vi "IsUserInputInRange.vi"(11 "User Input in":T1) -> (3 "InRange?":bool)   [LabVIEW 2017]
uses:
  Ctrl/UserInput.ctl
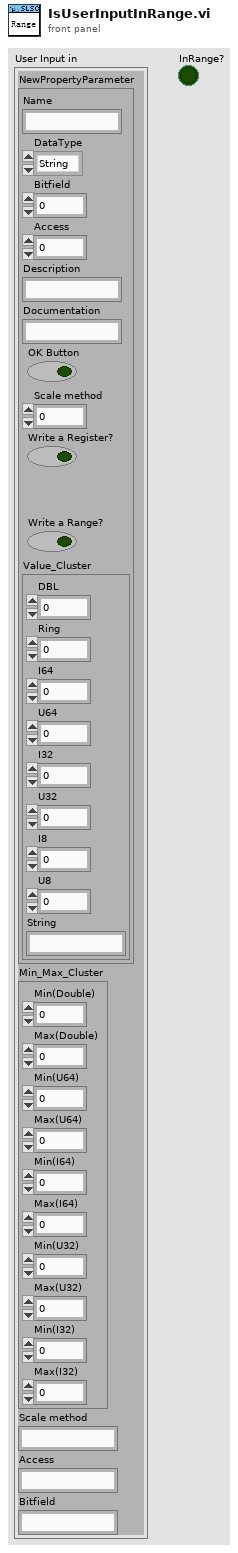
[diagram p1: front panel]
types:
  T1 = typedef "UserInput.ctl" = cluster{"NewPropertyParameter":cluster{"Name":string, "DataType":enum16{"String", "Double", "U64", "I64", "U32", "I32", "Bool"}, "Bitfield":u16, "Access":u16, "Description":string, "Documentation":string, "OK Button":bool, "Scale method":u16, "Write a Register?":bool, "Write a Range?":bool, "Value_Cluster":cluster{"DBL":dbl, "Ring":u16, "I64":i64, "U64":u64, "I32":i32, "U32":u32, "I8":i8, "U8":u8, "String":string}}, "Min_Max_Cluster":cluster{"Min(Double)":dbl, "Max(Double)":dbl, "Min(U64)":u64, "Max(U64)":u64, "Min(I64)":i64, "Max(I64)":i64, "Min(U32)":u32, "Max(U32)":u32, "Min(I32)":i32, "Max(I32)":i32}, "Scale method":string, "Access":string, "Bitfield":string}
  T2 = cluster{"DBL":dbl, "Ring":u16, "I64":i64, "U64":u64, "I32":i32, "U32":u32, "I8":i8, "U8":u8, "String":string}
  T3 = enum16{"String", "Double", "U64", "I64", "U32", "I32", "Bool"}
  T4 = cluster{"Min(Double)":dbl, "Max(Double)":dbl, "Min(U64)":u64, "Max(U64)":u64, "Min(I64)":i64, "Max(I64)":i64, "Min(U32)":u32, "Max(U32)":u32, "Min(I32)":i32, "Max(I32)":i32}
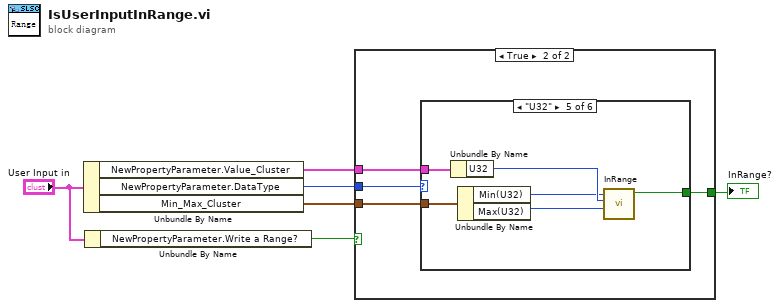
[diagram p0: block diagram]
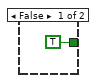
[diagram p2: hidden frame]
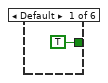
[diagram p3: hidden frame]
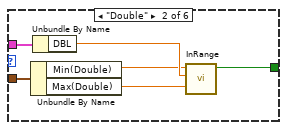
[diagram p4: hidden frame]
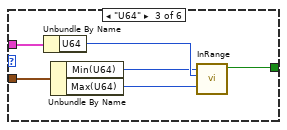
[diagram p5: hidden frame]
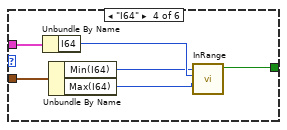
[diagram p6: hidden frame]
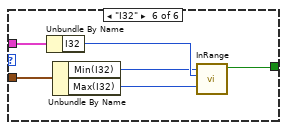
[diagram p7: hidden frame]
diagram:
  n1 = Unbundle By Name("User Input in") -> ("NewPropertyParameter.Value_Cluster"=w6:T2, "NewPropertyParameter.DataType"=w4:T3, "Min_Max_Cluster"=w5:T4)
  n2 = Unbundle By Name("User Input in") -> ("NewPropertyParameter.Write a Range?"=w1:bool)
  n3 = case shown="True" w1 {
    tunnel: w6 -> [_ w11]
    tunnel: w5 -> [_ w10]
    tunnel: w4 -> [_ w9]
    tunnel: [TRUE ("Boolean") w8] -> w2
    frame False {
    }
    frame True {
      n4 = case shown="\"U32\"" w9 {
        tunnel: w10 -> [_ w17 w22 w28 w34 w40]
        tunnel: w11 -> [_ w18 w23 w29 w35 w41]
        tunnel: [TRUE ("Boolean") w15 w21 w27 w33 w39] -> w8
        frame Default {
        }
        frame "Double" {
          n5 = Unbundle By Name(w17) -> ("Min(Double)"=w14:dbl, "Max(Double)"=w13:dbl)
          n6 = Unbundle By Name(w18) -> ("DBL"=w16:dbl)
          n7 = call "InRange.vi"("Max"=w13, "Value"=w16, "Min"=w14) -> ("Boolean"=w15:bool)  [unwired: 8 in]
        }
        frame "U64" {
          n8 = Unbundle By Name(w23) -> ("U64"=w24:u64)
          n9 = Unbundle By Name(w22) -> ("Min(U64)"=w19:u64, "Max(U64)"=w20:u64)
          n10 = call "InRange.vi"("Max"=w20, "Value"=w24, "Min"=w19) -> ("Boolean"=w21:bool)  [unwired: 8 in]
        }
        frame "I64" {
          n11 = Unbundle By Name(w29) -> ("I64"=w30:i64)
          n12 = Unbundle By Name(w28) -> ("Min(I64)"=w26:i64, "Max(I64)"=w25:i64)
          n13 = call "InRange.vi"("Max"=w25, "Value"=w30, "Min"=w26) -> ("Boolean"=w27:bool)  [unwired: 8 in]
        }
        frame "U32" {
          n14 = Unbundle By Name(w35) -> ("U32"=w36:u32)
          n15 = Unbundle By Name(w34) -> ("Min(U32)"=w32:u32, "Max(U32)"=w31:u32)
          n16 = call "InRange.vi"("Max"=w31, "Value"=w36, "Min"=w32) -> ("Boolean"=w33:bool)  [unwired: 8 in]
        }
        frame "I32" {
          n17 = Unbundle By Name(w41) -> ("I32"=w42:i32)
          n18 = Unbundle By Name(w40) -> ("Min(I32)"=w38:i32, "Max(I32)"=w37:i32)
          n19 = call "InRange.vi"("Max"=w37, "Value"=w42, "Min"=w38) -> ("Boolean"=w39:bool)  [unwired: 8 in]
        }
      }
    }
  }
  "InRange?" <- w2
